vi "ZM-CM-releaseProtocol.vi"(8 "error in (no error)":errorcluster, 11 "ZM-CM-communication_manager in":refnum<class "ZM-CM-communication_manager.lvclass">) -> (0 "error out":errorcluster, 3 "ZM-CM-communication_manager out":refnum<class "ZM-CM-communication_manager.lvclass">)   [LabVIEW 2020, in "ZM-CM-communication_manager.lvlib" / "ZM-CM-communication_manager.lvclass"]
doc: "Closes the communication manager's protocol (ZM-CP-close), called by Stop Core and after a failed init. Code 1 (a resource never opened) is cleared without a log; any other close error is logged with ZM-CU-log and passed on in error out."
uses:
  ZM-CM-communication_manager.lvclass
  ZM-CM-communication_manager.lvclass/ZM-CM-communication_manager.ctl
  protocol/ZM-CP-communication_protocol/ZM-CP-communication_protocol/ZM-CP-communication_protocol.lvclass
  common/ZM-CU-common_utilities/ZM-CU-common_utilities.lvlib
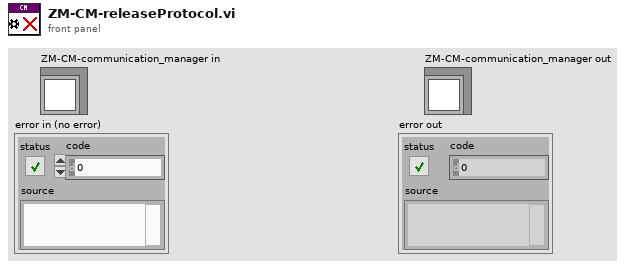
[diagram p1: front panel]
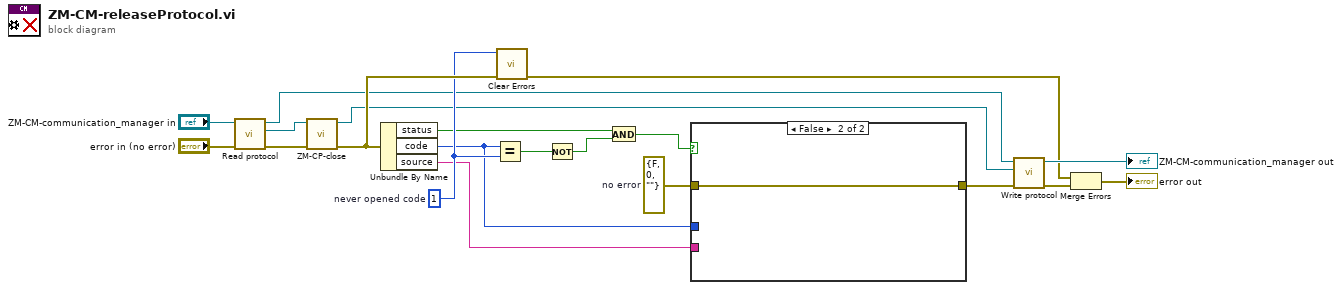
[diagram p0: block diagram]
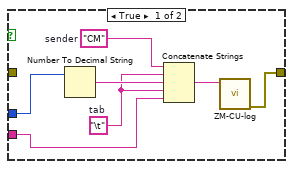
[diagram p2: hidden frame]
diagram:
  w9 = errorcluster {"status"=FALSE, "code"=0, "source"=""}  # no error
  w15 = 1  # never opened code
  n1 = call "Read protocol.vi"("error in (no error)"="error in (no error)", "ZM-CM-communication_manager in"="ZM-CM-communication_manager in") -> ("error out"=w17:errorcluster, "ZM-CP-communication_protocol.lvlib:ZM-CP-communication_protocol.lvclass"=w18:refnum<class "ZM-CP-communication_protocol.lvclass">, "ZM-CM-communication_manager out"=w6:refnum<class "ZM-CM-communication_manager.lvclass">)  [unwired: 7 in]
  n2 = call-dynamic "ZM-CP-close.vi"("error in (no error)"=w17, "ZM-CP-communication_protocol in"=w18) -> ("error out"=w16:errorcluster, "ZM-CP-communication_protocol out"=w5:refnum<class "ZM-CP-communication_protocol.lvclass">)  [unwired: 8 in]
  n3 = Unbundle By Name(w16) -> ("status"=w13:bool, "code"=w11:i32, "source"=w10:string)
  n4 = Equal?(x=w11, y=w15) -> (x = y?=w14:bool)
  n5 = call <vilib>:"Clear Errors.vi"("error in (no error)"=w16, "specific error code to clear (0: all)"=w15) -> ("error out"=w3:errorcluster)  [unwired: 4 in, 1 out]
  n6 = Not(x=w14) -> (.not. x?=w12:bool)
  n7 = And(x=w13, y=w12) -> (x .and. y?=w8:bool)
  n8 = case shown="False" w8 {
    tunnel: w11 -> [w27 _]
    tunnel: w10 -> [w23 _]
    tunnel: w9 -> [_ w28]
    tunnel: [w21 w28] -> w7
    frame True {
      w24 = "\t"  # tab
      w26 = "CM"  # sender
      n9 = Number To Decimal String(number=w27) -> (decimal integer string=w25:string)  [unwired: 1 in]
      n10 = Concatenate Strings(w26, w24, w25, w24, w23) -> (w22:string)
      n11 = call "ZM-CU-log.vi"("message"=w22) -> ("error out"=w21:errorcluster)  [unwired: 10 in]
    }
    frame False {
    }
  }
  n12 = call "Write protocol.vi"("error in (no error)"=w7, "ZM-CP-communication_protocol.lvlib:ZM-CP-communication_protocol.lvclass"=w5, "ZM-CM-communication_manager in"=w6) -> ("error out"=w2:errorcluster, "ZM-CM-communication_manager out"=→"ZM-CM-communication_manager out":refnum<class "ZM-CM-communication_manager.lvclass">)  [unwired: 7 in]
  n13 = Merge Errors(w3, w2) -> (→"error out":errorcluster)
